vi "SaveCFG.vi"(7 "Clear Before Saving(F)":bool, 8 "error in (no error)":errorcluster, 11 "object in":refnum<class "Template_CFG.lvclass">) -> (0 "error out":errorcluster, 2 "OK?":bool, 3 "object out":refnum<class "Template_CFG.lvclass">)   [LabVIEW 2021, in "Template-Channels.lvlib" / "Template_CFG.lvclass"]
doc: "Saves Configuration"
uses:
  Template_CFG.lvclass
  C:/Users/averna/Documents/LV Gym DEMO/Factory Pattern/Channels/Dependencies/Channel.lvlibp/Channel/Configuration_class/Configuration.lvclass
  Dependencies/Channel.lvlibp/Channel/Configuration_class/properties/ReadConfigurationFile.vi
  <vilib>/Utility/config.llb/Write Key (String).vi
  <vilib>/Utility/config.llb/Write Key (I32).vi
  Dependencies/Channel.lvlibp/Channel/Configuration_class/Configuration.lvclass
  <vilib>/Utility/config.llb/NI_LVConfig.lvlib
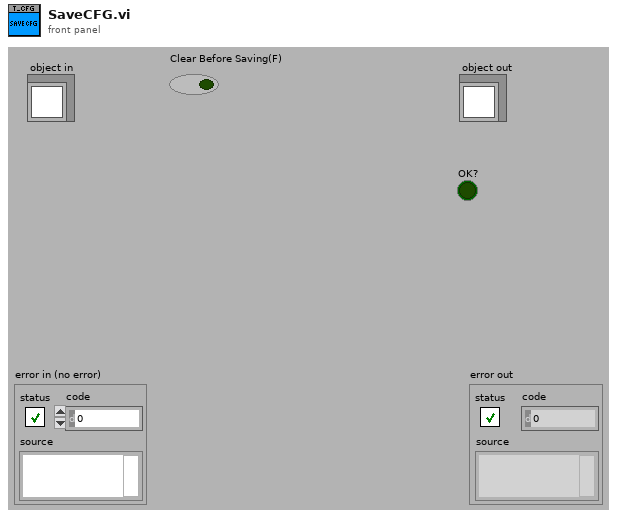
[diagram p1: front panel]
types:
  T1 = typedef "NI_LVConfig.lvlib/Config Data RefNum.ctl" = refnum<k1>
  T2 = typedef "Template-Channels.lvlib/Template_CFG.lvclass/Data.ctl" = cluster{"Alias":string}
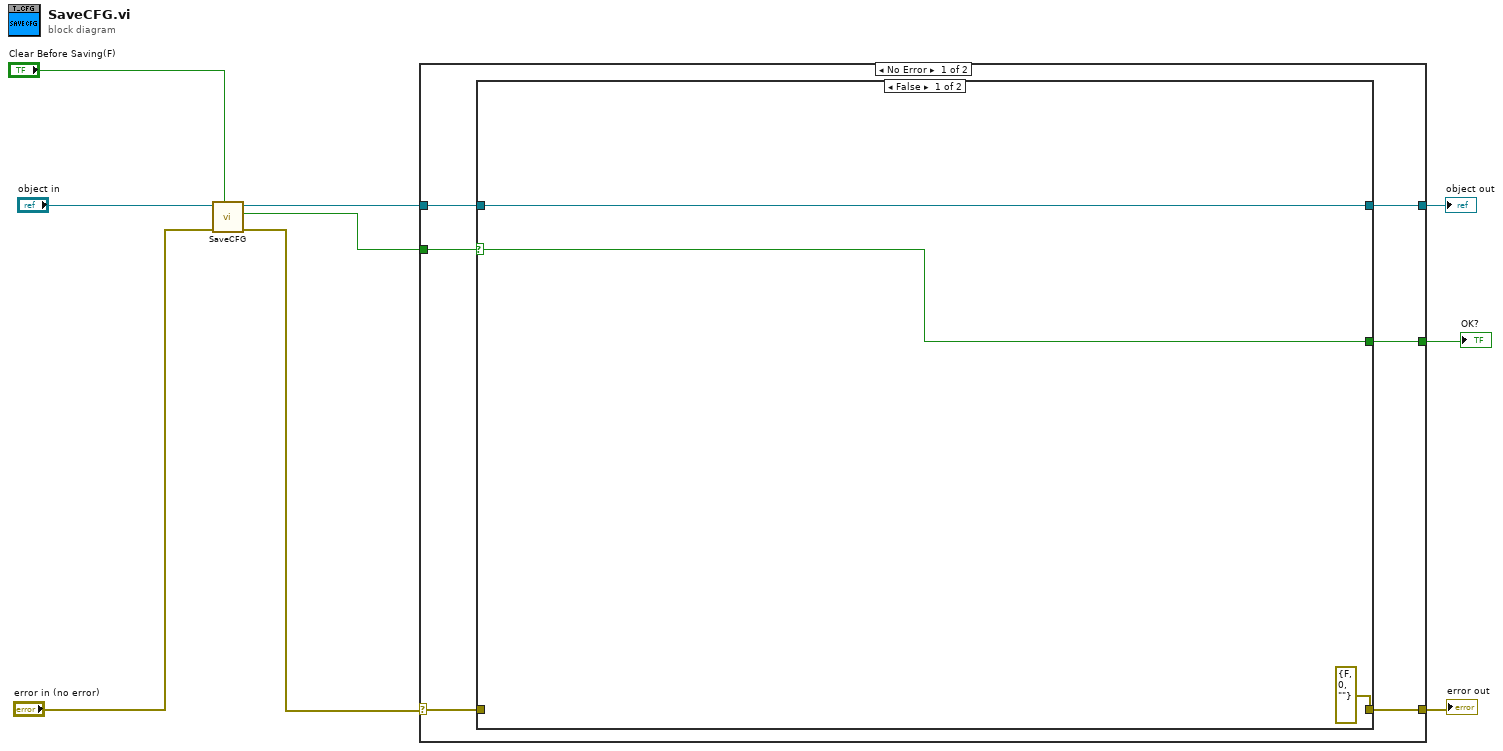
[diagram p0: block diagram]
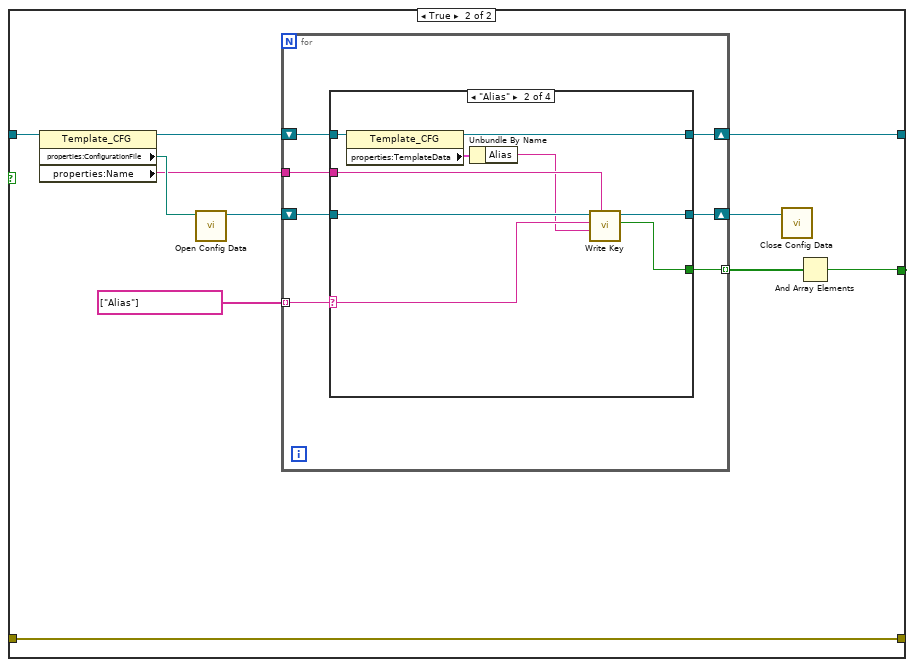
[diagram p2: hidden frame]
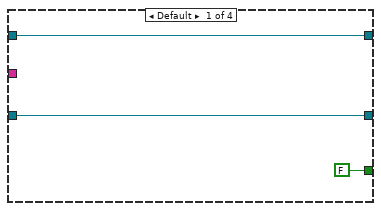
[diagram p3: hidden frame]
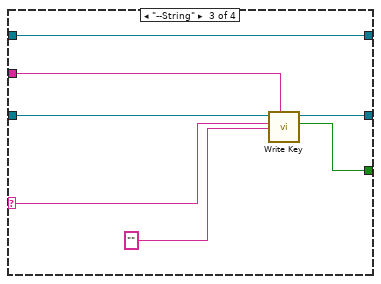
[diagram p4: hidden frame]
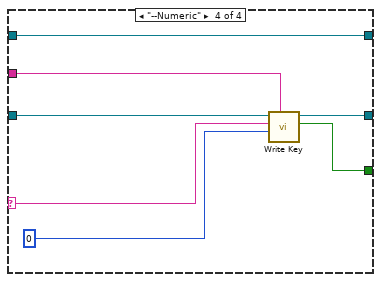
[diagram p5: hidden frame]
diagram:
  n1 = call-parent "SaveCFG.vi"("Clear Before Saving(F)"="Clear Before Saving(F)", "error in (no error)"="error in (no error)", "object in"="object in") -> ("error out"=w5:errorcluster, "OK?"=w3:bool, "object out"=w7:refnum<class "Template_CFG.lvclass">)  [unwired: 6 in]
  n2 = case shown="No Error" w5 {
    selector: w5 -> [w12 w65]
    tunnel: [w13 w65] -> w9
    tunnel: w7 -> [w14 w64]
    tunnel: [w10 w63] -> w2
    tunnel: w3 -> [w11 w63]
    tunnel: [w15 w64] -> w1
    frame No Error {
      n3 = case shown="False" w11 {
        selector: w11 -> [w17 _]
        tunnel: [w18 w25] -> w15
        tunnel: w14 -> [w18 w29]
        tunnel: [errorcluster {"status"=FALSE, "code"=0, "source"=""} ("error IO") w28] -> w13
        tunnel: w12 -> [_ w28]
        tunnel: [w17 w19] -> w10
        frame False {
        }
        frame True {
          n4 = property class="Template_CFG"(reference=w29) -> (reference out=w24:refnum<class "Template_CFG.lvclass">, "properties:ConfigurationFile"=w27:path, "properties:Name"=w21:string)  [unwired: 1 in, 1 out]
          n5 = call <vilib>:"Open Config Data.vi"("configuration file path"=w27) -> ("refnum"=w26:T1)  [unwired: 8 in, 2 out]
          n6 = for {
            shift-right: [w32] -> w25
            shift-left: w24 -> [w31]
            shift-right: [w35] -> w23
            shift-left: w26 -> [w36]
            tunnel: string[] ["Alias"] -> [w34] mode=indexing
            tunnel: w21 -> [w33]
            tunnel: [w30] -> w20 mode=indexing
            n7 = case shown="\"Alias\"" w34 {
              selector: w34 -> [_ w46 w53 w57]
              tunnel: w36 -> [w38 w48 w55 w62]
              tunnel: [w38 w47 w54 w61] -> w35
              tunnel: w33 -> [_ w45 w52 w60]
              tunnel: [w39 w43 w51 w59] -> w32
              tunnel: w31 -> [w39 w44 w51 w59]
              tunnel: [FALSE ("found?") w40 w49 w56] -> w30
              frame Default {
              }
              frame "Alias" {
                n8 = property class="Template_CFG"(reference=w44) -> (reference out=w43:refnum<class "Template_CFG.lvclass">, "properties:TemplateData"=w42:T2)  [unwired: 1 in, 1 out]
                n9 = Unbundle By Name(w42) -> ("Alias"=w41:string)
                n10 = call-poly <vilib>:"Write Key.vi"("section"=w45, "value"=w41, "key"=w46, "refnum"=w48) -> ("found?"=w40:bool, "refnum out"=w47:T1)  [unwired: 5 in, 1 out]
              }
              frame "--String" {
                n11 = call-poly <vilib>:"Write Key.vi"("section"=w52, "value"="", "key"=w53, "refnum"=w55) -> ("found?"=w49:bool, "refnum out"=w54:T1)  [unwired: 5 in, 1 out]
              }
              frame "--Numeric" {
                n12 = call-poly <vilib>:"Write Key.vi"("section"=w60, "value"=0, "key"=w57, "refnum"=w62) -> ("found?"=w56:bool, "refnum out"=w61:T1)  [unwired: 5 in, 1 out]
              }
            }
          }
          n13 = call <vilib>:"Close Config Data.vi"("refnum"=w23) -> ()  [unwired: 9 in, 2 out]
          n14 = And Array Elements(Boolean array=w20) -> (logical AND=w19:bool)
        }
      }
    }
    frame Error {
    }
  }
  "error out" <- w9
  "object out" <- w1
  "OK?" <- w2
